vi "DAC Save Results.vi"(8 "error in":errorcluster, 9 "Log Details?":bool, 10 "tdms file":refnum<k34>, 11 "DAC HMP4040 in":refnum<class "DAC HMP4040.lvclass">) -> (0 "error out":errorcluster)   [LabVIEW 2019, in "DAC.lvlib" / "DAC HMP4040.lvclass"]
uses:
  DAC HMP4040.lvclass
  DAC.lvclass
  C:/Users/krio/Documents/LV_Projects/test-stand/App/DAC/DAC.lvclass
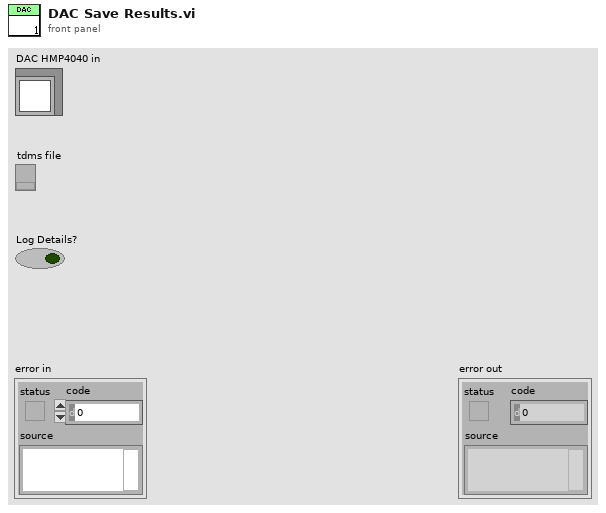
[diagram p1: front panel]
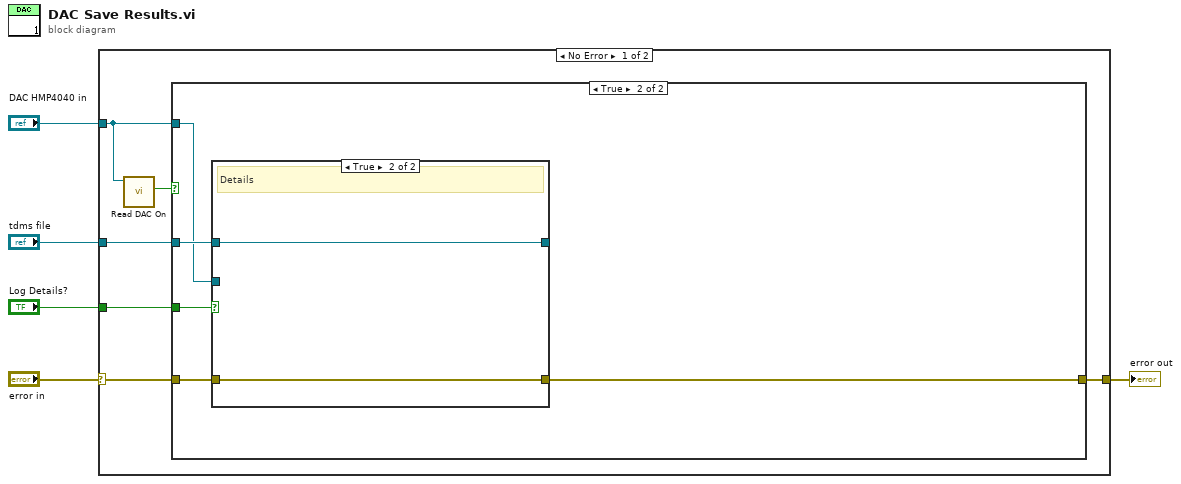
[diagram p0: block diagram]
diagram:
  n1 = case shown="No Error" "error in" {
    selector: "error in" -> [w6 w22]
    tunnel: "DAC HMP4040 in" -> [w11 _]
    tunnel: "tdms file" -> [w9 _]
    tunnel: [w8 w22] -> w2
    tunnel: "Log Details?" -> [w7 _]
    frame No Error {
      n2 = call "Read DAC On.vi"("DAC in"=w11) -> ("DAC On"=w10:bool)  [unwired: 8 in, 2 out]
      n3 = case shown="True" w10 {
        tunnel: w11 -> [_ w14]
        tunnel: w9 -> [_ w16]
        tunnel: [w12 w13] -> w8
        tunnel: w7 -> [_ w17]
        tunnel: w6 -> [w12 w15]
        frame False {
        }
        frame True {
          n4 = case shown="True" w17 {
            tunnel: w16 -> [w19 w21]
            tunnel: [w19 w21] -> _
            tunnel: w14 -> [_ _]
            tunnel: w15 -> [w18 w20]
            tunnel: [w18 w20] -> w13
            frame False {
            }
            frame True {
              # "Details"
            }
          }
        }
      }
    }
    frame Error {
    }
  }
  "error out" <- w2
